vi "RemoteVI Launch Server Loop.vi"(0 "Server Loop":refnum<vi>, 1 "stop notifier name":string, 2 "share":T1, 5 "VI":refnum<vi>, 7 "port":u16=8088, 9 "fps":dbl=20.0, 11 "error in":errorcluster) -> (15 "error out":errorcluster)   [LabVIEW 2020, in "RemoteVI.lvlib"]
doc: "Runs RemoteVI Server Loop.vi asynchronously and waits until it listens: sets its controls (RemoteVI Set Server Loop Inputs.vi), obtains the notifier <stop notifier name>:started, runs the loop without waiting and with Auto Dispose Ref, and waits up to 2 s for the loop's listener result. error out is that result (e.g. 60 when the port is in use - the loop has then already ended), 5002 when nothing arrived within 2 s, or an error of setting the controls or running the loop."
uses:
  RemoteVI.lvlib
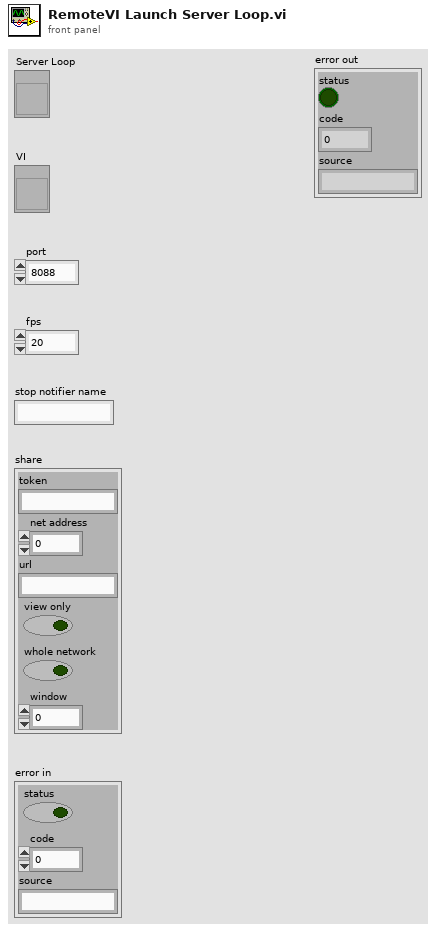
[diagram p1: front panel]
types:
  T1 = cluster{"token":string, "net address":u32, "url":string, "view only":bool, "whole network":bool, "window":u64}
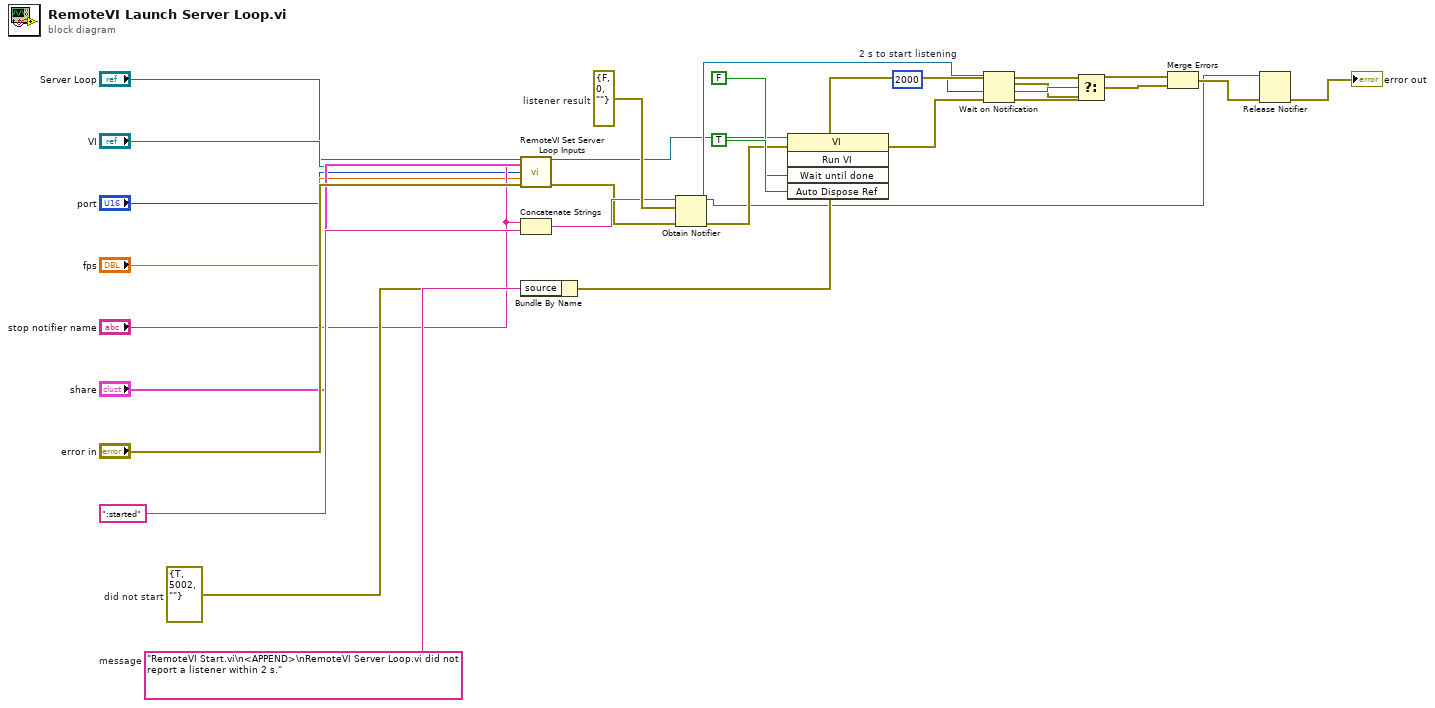
[diagram p0: block diagram]
diagram:
  w23 = "RemoteVI Start.vi\n<APPEND>\nRemoteVI Server Loop.vi did not report a listener within 2 s."  # message
  w22 = errorcluster {"status"=TRUE, "code"=5002, "source"=""}  # did not start
  w18 = 2000  # 2 s to start listening
  w12 = errorcluster {"status"=FALSE, "code"=0, "source"=""}  # listener result
  n1 = call "RemoteVI Set Server Loop Inputs.vi"("Server Loop"="Server Loop", "stop notifier name"="stop notifier name", "share"="share", "VI"="VI", "port"="port", "fps"="fps", "error in"="error in") -> ("Server Loop out"=w8:refnum<vi>, "error out"=w9:errorcluster)  [unwired: 7 in]
  n2 = Concatenate Strings("stop notifier name", ":started") -> (w11:string)
  n3 = Bundle By Name(cluster=w22, "source"=w23) -> (w24:errorcluster)
  n4 = Obtain Notifier(name (unnamed)=w11, notification data type=w12, error in (no error)=w9) -> (notifier out=w13:refnum<notifier>, error out=w14:errorcluster)  [unwired: 1 in, 1 out]
  n5 = invoke class="VI" method="Run VI"(reference=w8, error in=w14, "Wait until done"=FALSE, "Auto Dispose Ref"=TRUE) -> (error out=w17:errorcluster)  [unwired: 1 in, 4 out]
  n6 = Wait on Notification(notifier=w13, timeout in ms (-1)=w18, error in (no error)=w17) -> (notification=w19:errorcluster, timed out?=w20:bool, error out=w21:errorcluster)  [unwired: 1 in, 1 out]
  n7 = Select(t=w24, s=w20, f=w19) -> (s? t:f=w25:errorcluster)
  n8 = Merge Errors(w21, w25) -> (w26:errorcluster)
  n9 = Release Notifier(notifier=w13, error in (no error)=w26) -> (error out=→"error out":errorcluster)  [unwired: 1 in, 2 out]
